vi "Native_AddGrowableInDiagram.vi"() -> ()   [LabVIEW 2024]
panel:
  out "error out":errorcluster caption="错误输出"
  out "terminal_ids":u32[](array[numeric])
  in  "terminal_ids type":u32
  out "object_id":u32
  in  "object_id type":u32
  in  "y":i16=100
  in  "x":i16=100
  in  "style":u32
  in  "owner_diagram_id":u32
  in  "target_path":path
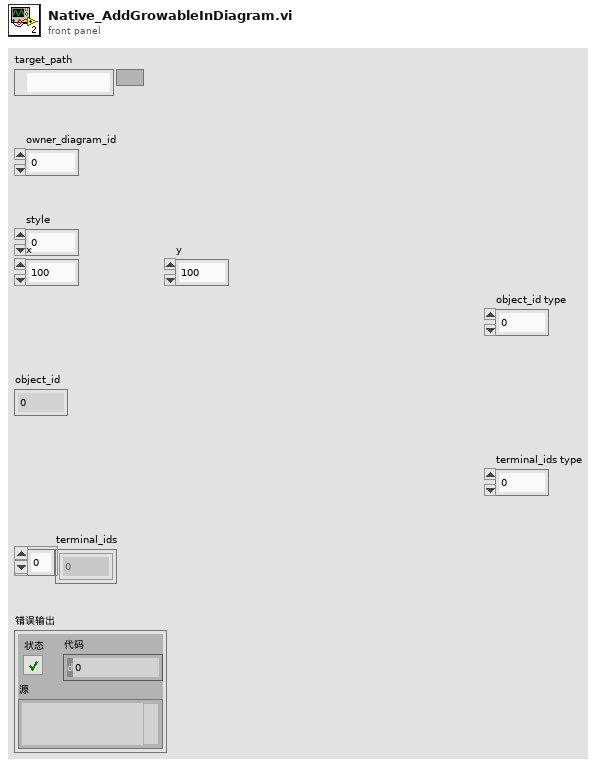
[diagram p1: front panel]
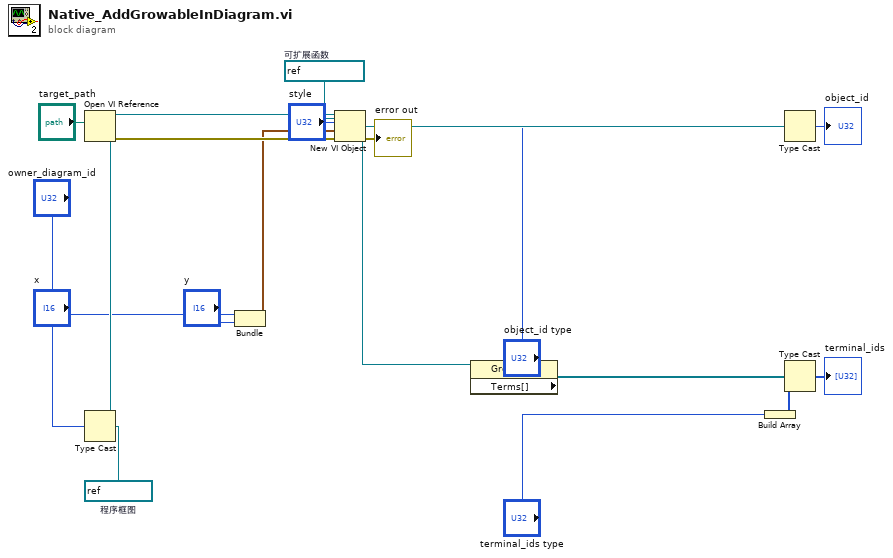
[diagram p0: block diagram]
diagram:
  w15 = refnum<vi> refnum  # 可扩展函数
  w16 = refnum<vi> refnum  # 程序框图
  n1 = Open VI Reference ("打开VI引用")(vi path="target_path") -> (error out=w13:errorcluster)  [unwired: 5 in, 1 out]
  n2 = Type Cast ("强制类型转换")(type=w16, x="owner_diagram_id") -> (*(type *) &x=w14:refnum<vi>)
  n3 = Bundle ("捆绑")("x"="x", "y"="y") -> (w9:cluster{"x":i16, "y":i16})  [unwired: 1 in]
  n4 = New VI Object ("新建VI对象")(vi object class=w15, owner refnum=w14, style="style", position/next to=w9, 8:w13) -> (object refnum=w8:refnum<vi>, 0:→"error out":errorcluster)  [unwired: 3 in]
  n5 = property on="属性节点" class="GrowFunc"(reference=w8) -> ("Terms[]"=w5:refnum<vi>[])  [unwired: 1 in, 2 out]
  n6 = Build Array ("创建数组")("terminal_ids type") -> (w3:u32[])
  n7 = Type Cast ("强制类型转换")(type="object_id type", x=w8) -> (*(type *) &x=→"object_id":u32)
  n8 = Type Cast ("强制类型转换")(type=w3, x=w5) -> (*(type *) &x=→"terminal_ids":u32[])
